vi "RDB Send Message.vi"(8 "error in (no error)":errorcluster, 11 "Settings in":T1={"UDP Receiver"=refnum, "UDP Sender"=refnum, "Valid Packet"=FALSE, "TCP"=refnum, "Network Settings"={"IP adress"="127.0.0.1", "RDB"={"Protocol"=enum."UDP", "Tx Port"=48270, "Rx Port"=10, "Buffer Size"=204800, "Timeout"=10}, "SCP"={"Protocol"=enum."TCP", "Tx Port"=48191, "Rx Port"=48191, "Buffer Size"=204800, "Timeout"=10}}, "vclient"=path "", "paeseHandle"=0, "builderHandle"=0}) -> (0 "error out":errorcluster, 1 "RDB Message":string, 3 "Settings out":T1={"UDP Receiver"=refnum, "UDP Sender"=refnum, "Valid Packet"=FALSE, "TCP"=refnum, "Network Settings"={"IP adress"="127.0.0.1", "RDB"={"Protocol"=enum."UDP", "Tx Port"=48270, "Rx Port"=10, "Buffer Size"=204800, "Timeout"=10}, "SCP"={"Protocol"=enum."TCP", "Tx Port"=48191, "Rx Port"=48191, "Buffer Size"=204800, "Timeout"=10}}, "vclient"=path "", "paeseHandle"=0, "builderHandle"=0})   [LabVIEW 2023, in "RDB.lvlib"]
uses:
  RDB.lvlib
  Engine/Type/Settings.ctl
  Shared/Network Settings.ctl
  Shared/Protocol.ctl
  Shared/Vires VTD Shared.lvlib
  Engine/Vires VTD Engine.lvlib
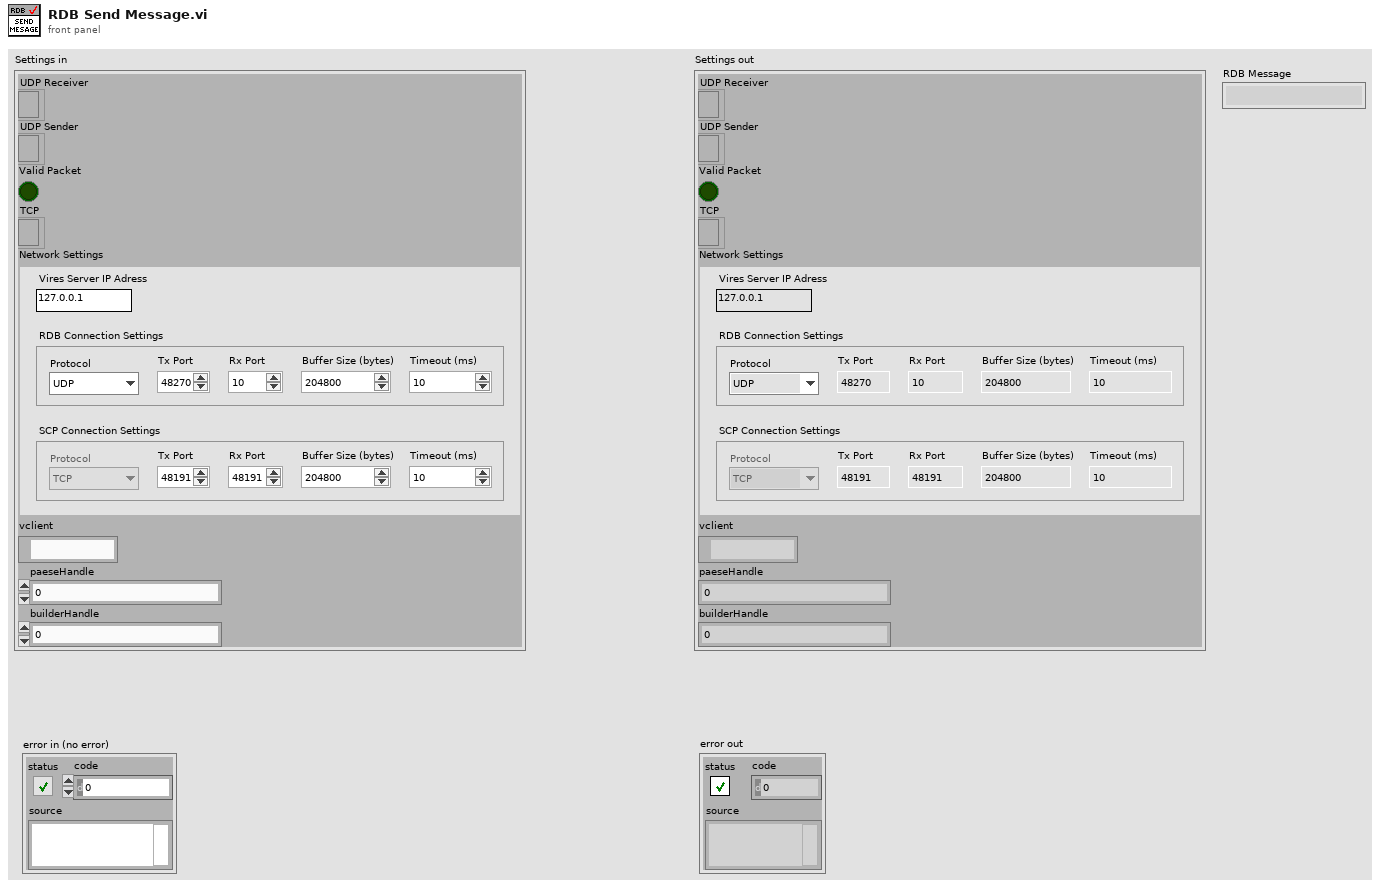
[diagram p1: front panel]
types:
  T1 = typedef "Vires VTD Engine.lvlib/Settings.ctl" = cluster{"UDP Receiver":refnum<k16>, "UDP Sender":refnum<k16>, "Valid Packet":bool, "TCP":refnum<k5>, "Network Settings":T2, "vclient":path, "paeseHandle":u64, "builderHandle":u64}
  T2 = typedef "Vires VTD Shared.lvlib/Network Settings.ctl" = cluster{"IP adress":string, "RDB":cluster{"Protocol":T3, "Tx Port":u16, "Rx Port":u16, "Buffer Size":i32, "Timeout":u16}, "SCP":cluster{"Protocol":T3, "Tx Port":u16, "Rx Port":u16, "Buffer Size":i32, "Timeout":u16}}
  T3 = typedef "Vires VTD Shared.lvlib/Protocol.ctl" = enum16{"UDP", "TCP"}
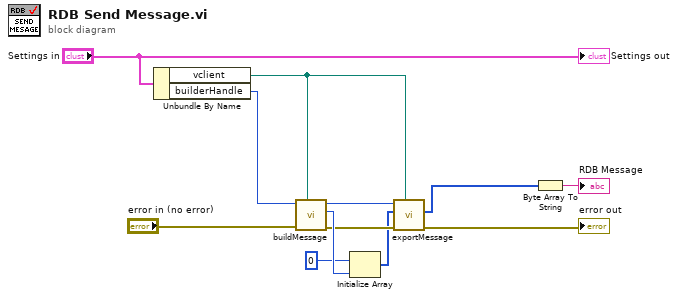
[diagram p0: block diagram]
diagram:
  n1 = Unbundle By Name("Settings in") -> ("vclient"=w11:path, "builderHandle"=w9:u64)
  n2 = call "buildMessage.vi"("path in"=w11, "error in (no error)"="error in (no error)", "builderHandle in"=w9) -> ("error out"=w5:errorcluster, "pMessageSize"=w8:i32, "builderHandle out"=w10:u64)  [unwired: 6 in]
  n3 = Initialize Array(u8 0, w8) -> (w3:u8[])
  n4 = call "exportMessage.vi"("path in"=w11, "error in (no error)"=w5, "dataOut"=w3, "builderHandle in"=w10) -> ("error out"=→"error out":errorcluster, "dataOut"=w2:u8[])  [unwired: 5 in, 1 out]
  n5 = Byte Array To String(unsigned byte array=w2) -> (string=→"RDB Message":string)
  "Settings out" <- "Settings in"
